vi "EDWARDS.vi"() -> ()   [LabVIEW 2022 SP3]
uses:
  Enum/Enum p4.ctl
  Variables globales/Variable glob generale.vi
  Variables globales/Variable glob Edwards.vi
  <vilib>/Instr/_visa.llb/VISA Configure Serial Port (Instr).vi
panel:
  out "Grappes TIC":cluster{"TIC":u8, "Voie":u8}[][](array[cluster])
  out "Sélection":bool[][](array[boolean])
  out "Port RS232 Edwards":refnum<visa-resource-name>[](array[refnum])
  out "Voies":i8[][](array[numeric]) min=1 max=6 step=1
  out "Données 1D":string[](array[string])
  out "Données Edwards":string[][](array[string])
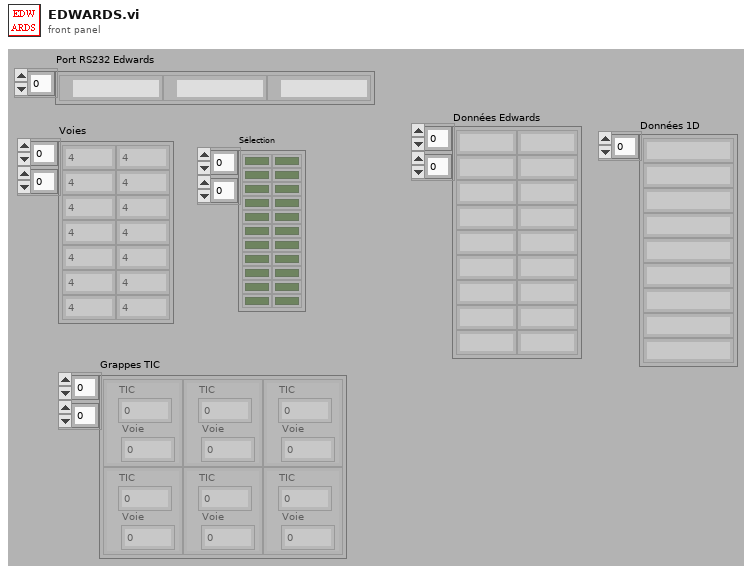
[diagram p1: front panel]
types:
  T1 = typedef "Enum p4.ctl" = enum16{"Init COM", "Lecture", "Grappes"}
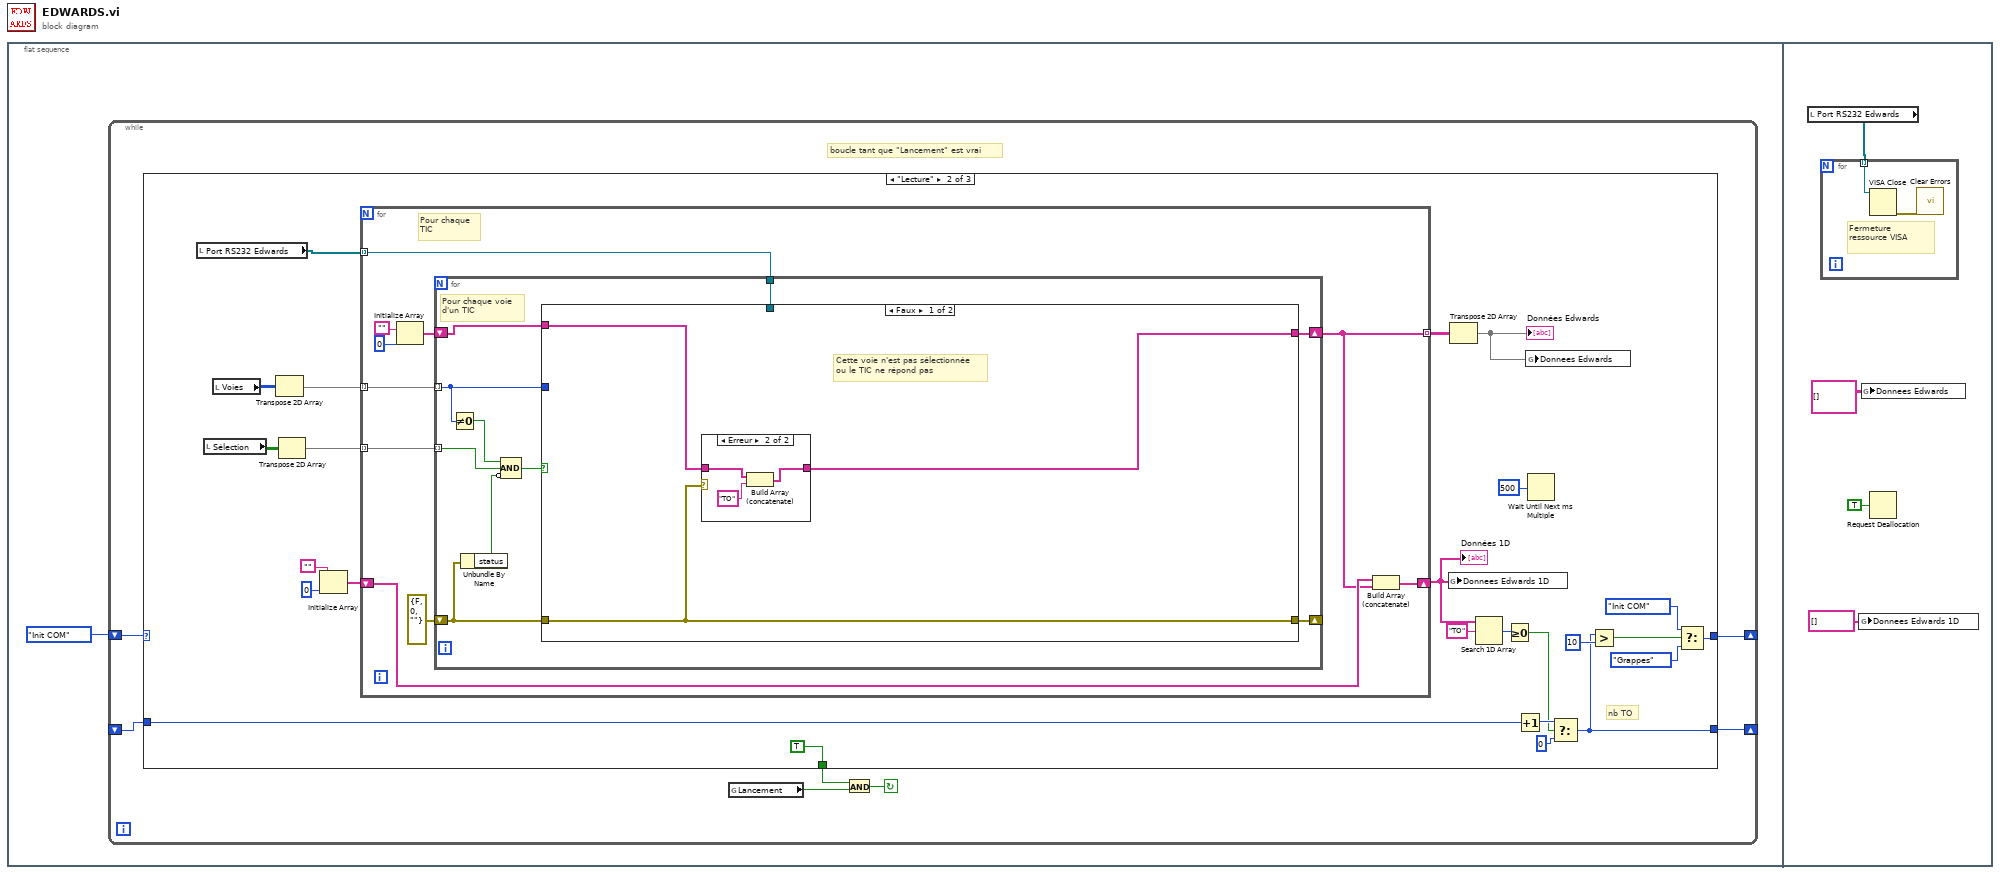
[diagram p0: block diagram]
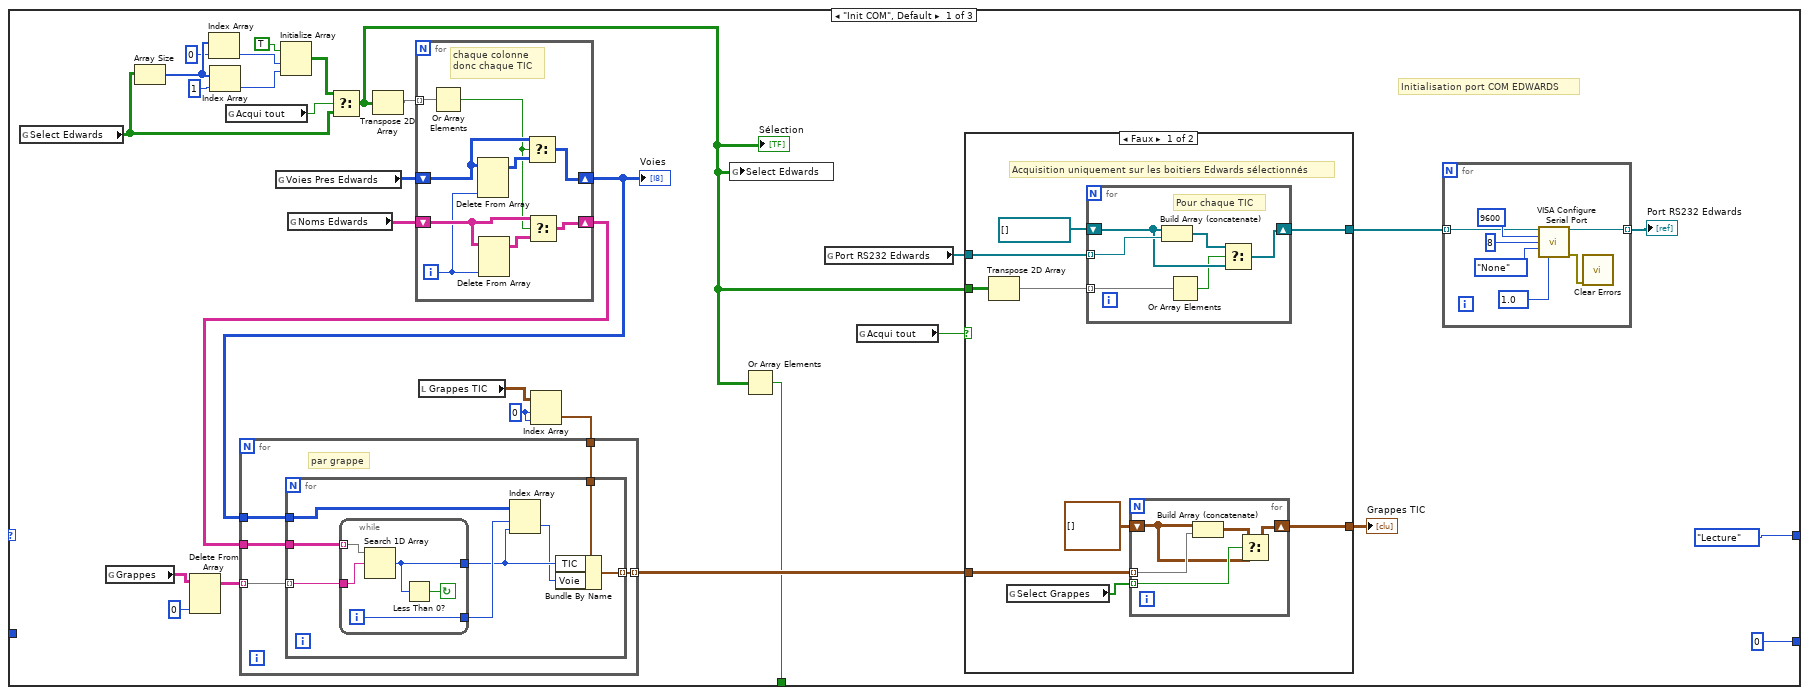
[diagram p2: hidden frame]
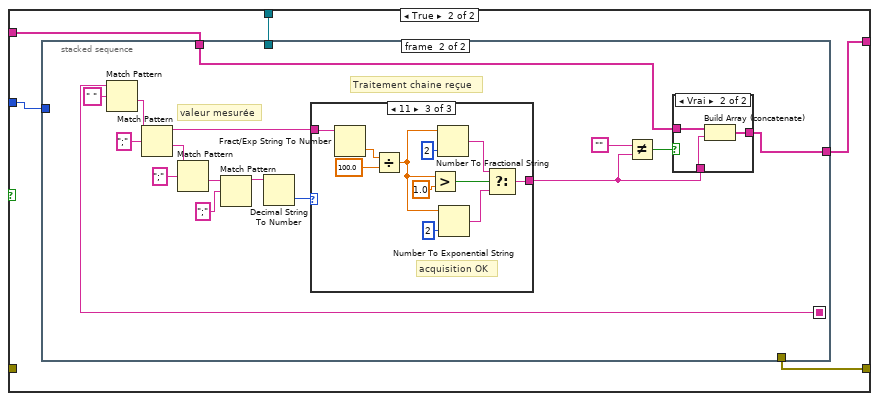
[diagram p5: hidden frame]
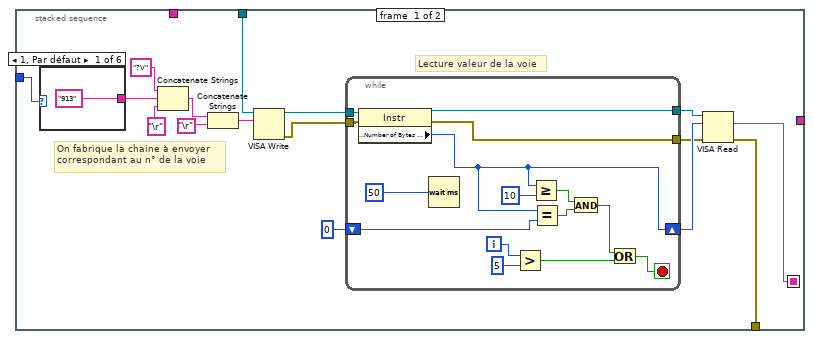
[diagram p6: hidden frame]
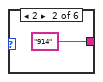
[diagram p7: hidden frame]
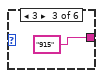
[diagram p8: hidden frame]
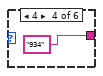
[diagram p9: hidden frame]
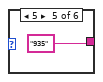
[diagram p10: hidden frame]
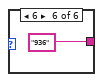
[diagram p11: hidden frame]
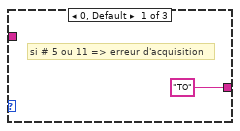
[diagram p13: hidden frame]
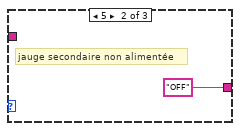
[diagram p14: hidden frame]
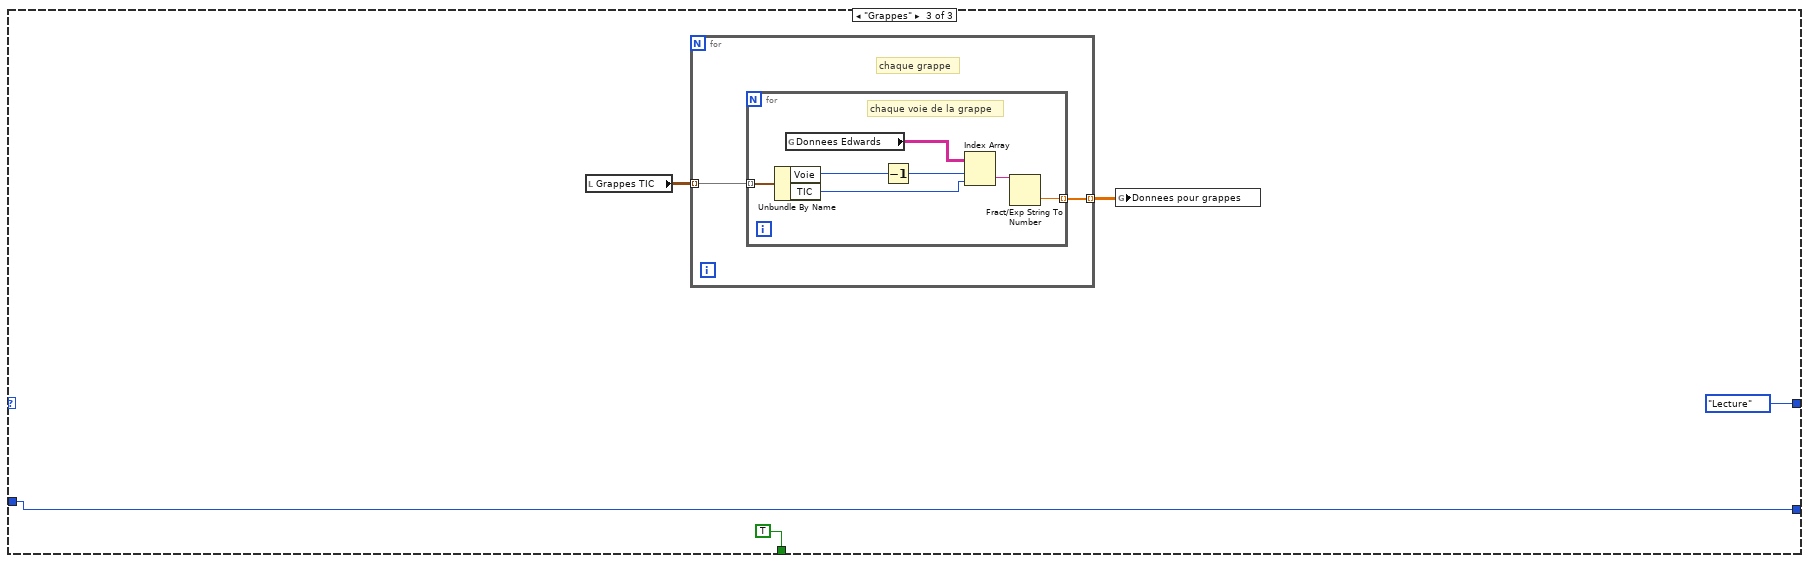
[diagram p15: hidden frame]
diagram:
  n1 = flat-sequence {
    frame #0 {
      n2 = while {
        shift-right: [w7] -> _
        shift-left: Enum_p4."Init COM" ("Énum") -> [w8]
        shift-right: [w6] -> _
        shift-left: _ -> [w5]
        stop <- w2 continue-if-true
        # "boucle tant que \"Lancement\" est vrai"
        n3 = case shown="\"Lecture\"" w8 {
          tunnel: [Enum_p4."Lecture" ("Énum") w104 Enum_p4."Lecture" ("Énum")] -> w7
          tunnel: [0 w100 w225] -> w6
          tunnel: w5 -> [_ w99 w225]
          tunnel: [w9 TRUE TRUE] -> w4
          frame "Init COM", Default {
            w24 = 0 ("indice (ligne)")
            # "Initialisation port COM EDWARDS"
            n4 = global read "Variable glob Edwards.vi" "Select Edwards"() -> (w19:bool[][])
            n5 = global read "Variable glob Edwards.vi" "Grappes"() -> (w25:string[][])
            n6 = Array Size(array=w19) -> (size(s)=w18:i32[])
            n7 = Delete From Array(array=w25, index (col)=0 ("indice désactivé (col)")) -> (array with subset deleted=w27:string[][])  [unwired: 2 in, 1 out]
            n8 = Index Array(array=w18, index=0 ("indice")) -> (element=w15:i32)
            n9 = Index Array(array=w18, index=1 ("indice")) -> (element=w14:i32)
            n10 = global read "Variable glob generale.vi" "Acqui tout"() -> (w20:bool)
            n11 = global read "Variable glob Edwards.vi" "Voies Pres Edwards"() -> (w30:i8[][])
            n12 = Initialize Array(TRUE, w15, w14) -> (w12:bool[][])
            n13 = global read "Variable glob Edwards.vi" "Noms Edwards"() -> (w31:string[][])
            n14 = Select(t=w12, s=w20, f=w19) -> (s? t:f=w10:bool[][])
            "Sélection" <- w10
            n15 = Transpose 2D Array(2D array=w10) -> (transposed array=w32:bool[][])
            n16 = for {
              tunnel: w32 -> [w65] mode=indexing
              shift-right: [w62] -> w23
              shift-left: w31 -> [w63]
              shift-right: [w57] -> w11
              shift-left: w30 -> [w60]
              i -> [w58]
              # "chaque colonne\ndonc chaque TIC"
              n17 = Or Array Elements(Boolean array=w65) -> (logical OR=w59:bool)
              n18 = Delete From Array(array=w60, index (col)=w58) -> (array with subset deleted=w61:i8[][])  [unwired: 2 in, 1 out]
              n19 = Delete From Array(array=w63, index (col)=w58) -> (array with subset deleted=w64:string[][])  [unwired: 2 in, 1 out]
              n20 = Select(t=w60, s=w59, f=w61) -> (s? t:f=w57:i8[][])
              n21 = Select(t=w63, s=w59, f=w64) -> (s? t:f=w62:string[][])
            }
            "Voies" <- w11
            n22 = local read "Grappes TIC"() -> (w29:cluster{"TIC":u8, "Voie":u8}[][])
            n23 = Index Array(array=w29, index (row)=w24, index (col)=w24) -> (element=w28:cluster{"TIC":u8, "Voie":u8})
            n24 = for {
              tunnel: w27 -> [w43] mode=indexing
              tunnel: w23 -> [w42]
              tunnel: w11 -> [w41]
              tunnel: [w40] -> w22 mode=indexing
              tunnel: w28 -> [w39]
              # "par grappe"
              n25 = for {
                tunnel: w43 -> [w48] mode=indexing
                tunnel: w42 -> [w49]
                tunnel: w41 -> [w47]
                tunnel: [w51] -> w40 mode=indexing
                tunnel: w39 -> [w50]
                n26 = while {
                  tunnel: w49 -> [w55] mode=indexing
                  tunnel: w48 -> [w56]
                  tunnel: [w54] -> w45
                  tunnel: [w52] -> w46
                  i -> [w52]
                  stop <- w53 continue-if-true
                  n27 = Search 1D Array(1D array=w55, element=w56) -> (index of element=w54:i32)  [unwired: 1 in]
                  n28 = Less Than 0?(x=w54) -> (x < 0?=w53:bool)
                }
                n29 = Index Array(array=w47, index (row)=w46, index (col)=w45) -> (element=w44:i8)
                n30 = Bundle By Name(cluster=w50, "TIC"=w45, "Voie"=w44) -> (w51:cluster{"TIC":u8, "Voie":u8})
              }
            }
            n31 = global write "Variable glob Edwards.vi" "Select Edwards"(w10) -> ()
            n32 = Or Array Elements(Boolean array=w10) -> (logical OR=w9:bool)
            n33 = global read "Variable glob Edwards.vi" "Port RS232 Edwards"() -> (w36:refnum<visa-resource-name>[])
            n34 = global read "Variable glob generale.vi" "Acqui tout"() -> (w37:bool)
            n35 = case shown="Faux" w37 {
              tunnel: [w73 w87] -> w35
              tunnel: w36 -> [w74 w87]
              tunnel: w10 -> [w71 _]
              tunnel: w22 -> [w67 w86]
              tunnel: [w66 w86] -> w21
              frame False {
                # "Acquisition uniquement sur les boitiers Edwards sélectionnés"
                n36 = Transpose 2D Array(2D array=w71) -> (transposed array=w70:bool[][])
                n37 = global read "Variable glob Edwards.vi" "Select Grappes"() -> (w69:bool[])
                n38 = for {
                  tunnel: w74 -> [w85] mode=indexing
                  tunnel: w70 -> [w80] mode=indexing
                  shift-right: [w83] -> w73
                  shift-left: refnum<visa-resource-name>[] [] -> [w82]
                  # "Pour chaque TIC"
                  n39 = Build Array (concatenate)(w82, w85) -> (w84:refnum<visa-resource-name>[])
                  n40 = Or Array Elements(Boolean array=w80) -> (logical OR=w81:bool)
                  n41 = Select(t=w84, s=w81, f=w82) -> (s? t:f=w83:refnum<visa-resource-name>[])
                }
                n42 = for {
                  tunnel: w69 -> [w79] mode=indexing
                  shift-right: [w75] -> w66
                  shift-left: cluster{"TIC":u8, "Voie":u8}[][] [] -> [w76]
                  tunnel: w67 -> [w78] mode=indexing
                  n43 = Build Array (concatenate)(w76, w78) -> (w77:cluster{"TIC":u8, "Voie":u8}[][])
                  n44 = Select(t=w77, s=w79, f=w76) -> (s? t:f=w75:cluster{"TIC":u8, "Voie":u8}[][])
                }
              }
              frame True {
                # "Acquisition sur l'ensemble des boitiers Edwards configurés"
              }
            }
            "Grappes TIC" <- w21
            n45 = for {
              tunnel: w35 -> [w90] mode=indexing
              tunnel: [w89] -> w38 mode=indexing
              w94 = u16 10 items=["1.0"=10, "1.5"=15, "2.0"=20] ("stop bits (10: 1 bit)")
              n46 = call-poly "VISA Configure Serial Port"("VISA resource name"=w90, "baud rate (9600)"=u32 9600, "data bits (8)"=u16 8, "parity (0:none)"=enum16{"None", "Odd", "Even", "Mark", "Space"}."None", "stop bits (10: 1 bit)"=w94) -> ("VISA resource name out"=w89:refnum<visa-resource-name>, "error out"=w88:errorcluster)  [unwired: 9 in]
              n47 = call <vilib>:"Clear Errors.vi"("error in (no error)"=w88) -> ()  [unwired: 5 in, 2 out]
            }
            "Port RS232 Edwards" <- w38
          }
          frame "Lecture" {
            # "nb TO"
            n48 = local read "Port RS232 Edwards"() -> (w113:refnum<visa-resource-name>[])
            n49 = local read "Sélection"() -> (w96:bool[][])
            n50 = local read "Voies"() -> (w112:i8[][])
            n51 = Transpose 2D Array(2D array=w112) -> (transposed array=w111:i8[][])
            n52 = Transpose 2D Array(2D array=w96) -> (transposed array=w110:bool[][])
            n53 = Initialize Array("", 0 ("taille de la dimension")) -> (w116:string[])
            n54 = for {
              tunnel: w111 -> [w129] mode=indexing
              tunnel: [w122] -> w119 mode=indexing
              tunnel: w110 -> [w125] mode=indexing
              tunnel: w113 -> [w121] mode=indexing
              shift-right: [w123] -> w109
              shift-left: w116 -> [w124]
              # "Pour chaque\nTIC"
              n55 = Initialize Array("", 0 ("taille de la dimension")) -> (w126:string[])
              n56 = for {
                tunnel: w129 -> [w136] mode=indexing
                tunnel: w121 -> [w139]
                shift-right: [w138] -> w122
                shift-left: w126 -> [w137]
                tunnel: w125 -> [w133] mode=indexing
                shift-right: [w135] -> _
                shift-left: errorcluster {"status"=FALSE, "code"=0, "source"=""} ("error out") -> [w131]
                # "Pour chaque voie\nd'un TIC"
                n57 = Not Equal To 0?(x=w136) -> (x != 0?=w134:bool)
                n58 = Unbundle By Name(w131) -> ("status"=w130:bool)
                n59 = Compound Arithmetic op=AND ("Opérateur arithmétique")(w134, w133, invert w130) -> (w132:bool)
                n60 = case shown="Faux" w132 {
                  tunnel: w136 -> [_ w150]
                  tunnel: w139 -> [_ w151]
                  tunnel: [w140 w148] -> w138
                  tunnel: w137 -> [w141 w149]
                  tunnel: [w142 w147] -> w135
                  tunnel: w131 -> [w142 _]
                  frame False {
                    # "Cette voie n'est pas sélectionnée\nou le TIC ne répond pas"
                    n61 = case shown="Erreur" w142 {
                      tunnel: w141 -> [w143 w146]
                      tunnel: [w143 w145] -> w140
                      frame No Error {
                      }
                      frame Error {
                        n62 = Build Array (concatenate)(w146, "TO") -> (w145:string[])
                      }
                    }
                  }
                  frame True {
                    n63 = stacked-sequence {
                      seq-local: [w154 _] -> [_ w194]
                      tunnel: w151 -> [w158 _]
                      tunnel: w150 -> [w155 _]
                      tunnel: w149 -> [_ w191]
                      tunnel: [_ w189] -> w148
                      tunnel: [w152 _] -> w147
                      frame #0 {
                        # "Lecture valeur de la voie"
                        # "On fabrique la chaine à envoyer\ncorrespondant au n° de la voie"
                        n64 = case shown="1, Par défaut" w155 {
                          tunnel: ["913" "914" "915" "934" "935" "936"] -> w156
                          frame 1, Default {
                          }
                          frame 2 {
                          }
                          frame 3 {
                          }
                          frame 4 {
                          }
                          frame 5 {
                          }
                          frame 6 {
                          }
                        }
                        n65 = Concatenate Strings("?V", w156, "\r") -> (w160:string)
                        n66 = Concatenate Strings(w160, "\r") -> (w157:string)
                        n67 = VISA Write(VISA resource name=w158, write buffer=w157) -> (VISA resource name out=w163:refnum<visa-resource-name>, error out=w153:errorcluster)  [unwired: 1 in, 1 out]
                        n68 = while {
                          tunnel: w163 -> [w188]
                          tunnel: [w181] -> w167
                          shift-right: [w180] -> w166
                          shift-left: 0 -> [w179]
                          tunnel: w153 -> [w175]
                          tunnel: [w174] -> w159
                          i -> [w186]
                          stop <- w187 stop-if-true
                          n69 = property class="Instr"(reference=w188, error in=w175) -> (reference out=w181:refnum<visa-resource-name>, error out=w174:errorcluster, "Serial Settings:Number of Bytes at Serial Port"=w180:u32)
                          n70 = Wait (ms)(milliseconds to wait=u32 50 ("attente (ms)")) -> ()  [unwired: 1 out]
                          n71 = Greater?(x=w186, y=5) -> (0:w184:bool)
                          n72 = Greater Or Equal?(x=w180, y=u32 10) -> (x >= y?=w177:bool)
                          n73 = Equal?(x=w180, y=w179) -> (x = y?=w178:bool)
                          n74 = And(x=w177, y=w178) -> (x .and. y?=w176:bool)
                          n75 = Or(x=w176, y=w184) -> (x .or. y?=w187:bool)
                        }
                        n76 = VISA Read(VISA resource name=w167, byte count=w166, error in (no error)=w159) -> (read buffer=w154:string, error out=w152:errorcluster)  [unwired: 2 out]
                      }
                      frame #1 {
                        # "valeur mesurée"
                        # "Traitement chaine reçue"
                        n77 = Match Pattern(string=w194, regular expression=" " ("expression régulière")) -> (after substring=w196:string)  [unwired: 1 in, 3 out]
                        n78 = Match Pattern(string=w196, regular expression=";" ("expression régulière")) -> (before substring=w200:string, after substring=w199:string)  [unwired: 1 in, 2 out]
                        n79 = Match Pattern(string=w199, regular expression=";" ("expression régulière")) -> (after substring=w201:string)  [unwired: 1 in, 3 out]
                        n80 = Match Pattern(string=w201, regular expression=";" ("expression régulière")) -> (before substring=w203:string)  [unwired: 1 in, 3 out]
                        n81 = Decimal String To Number(string=w203) -> (number=w204:i32)  [unwired: 2 in, 1 out]
                        n82 = case shown="11" w204 {
                          tunnel: w200 -> [_ _ w221]
                          tunnel: ["TO" "OFF" w215] -> w190
                          frame 0, Default {
                            # "si # 5 ou 11 => erreur d'acquisition"
                          }
                          frame 5 {
                            # "jauge secondaire non alimentée"
                          }
                          frame 11 {
                            # "acquisition OK"
                            n83 = Fract/Exp String To Number(string=w221) -> (number=w220:dbl)  [unwired: 3 in, 1 out]
                            n84 = Divide(x=w220, y=100.0) -> (x/y=w212:dbl)
                            n85 = Greater?(x=w212, y=1.0) -> (0:w213:bool)
                            n86 = Number To Fractional String(number=w212, precision (6)=i16 2 ("précision (6)")) -> (F-format string=w216:string)  [unwired: 2 in]
                            n87 = Number To Exponential String(number=w212, precision (6)=i16 2 ("précision (6)")) -> (E-format string=w211:string)  [unwired: 2 in]
                            n88 = Select(t=w216, s=w213, f=w211) -> (s? t:f=w215:string)
                          }
                        }
                        n89 = Not Equal?(x="", y=w190) -> (x != y?=w193:bool)
                        n90 = case shown="Vrai" w193 {
                          tunnel: w191 -> [w205 w208]
                          tunnel: w190 -> [_ w207]
                          tunnel: [w205 w206] -> w189
                          frame False {
                          }
                          frame True {
                            n91 = Build Array (concatenate)(w208, w207) -> (w206:string[])
                          }
                        }
                      }
                    }
                  }
                }
              }
              n92 = Build Array (concatenate)(w124, w122) -> (w123:string[])
            }
            "Données 1D" <- w109
            n93 = global write "Variable glob Edwards.vi" "Donnees Edwards 1D"(w109) -> ()
            n94 = Transpose 2D Array(2D array=w119) -> (transposed array=w114:string[][])
            "Données Edwards" <- w114
            n95 = Search 1D Array(1D array=w109, element="TO" ("élément")) -> (index of element=w107:i32)  [unwired: 1 in]
            n96 = Greater Or Equal To 0?(x=w107) -> (x >= 0?=w97:bool)
            n97 = Increment(x=w99) -> (x+1=w101:i32)
            n98 = global write "Variable glob Edwards.vi" "Donnees Edwards"(w114) -> ()
            n99 = Wait Until Next ms Multiple(millisecond multiple=u32 500 ("n millisecondes")) -> ()  [unwired: 1 out]
            n100 = Select(t=w101, s=w97, f=0 ("cas faux")) -> (s? t:f=w100:i32)
            n101 = Greater?(x=w100, y=10) -> (0:w98:bool)
            n102 = Select(t=Enum_p4."Init COM" ("Énum"), s=w98, f=Enum_p4."Grappes" ("Énum")) -> (s? t:f=w104:T1)
          }
          frame "Grappes" {
            n103 = local read "Grappes TIC"() -> (w224:cluster{"TIC":u8, "Voie":u8}[][])
            n104 = for {
              tunnel: w224 -> [w228] mode=indexing
              tunnel: [w227] -> w223 mode=indexing
              # "chaque grappe"
              n105 = for {
                tunnel: w228 -> [w235] mode=indexing
                tunnel: [w230] -> w227 mode=indexing
                # "chaque voie de la grappe"
                n106 = Unbundle By Name(w235) -> ("Voie"=w233:u8, "TIC"=w232:u8)
                n107 = global read "Variable glob Edwards.vi" "Donnees Edwards"() -> (w234:string[][])
                n108 = Decrement(x=w233) -> (x-1=w229:u8)
                n109 = Index Array(array=w234, index (row)=w229, index (col)=w232) -> (element=w231:string)
                n110 = Fract/Exp String To Number(string=w231) -> (number=w230:dbl)  [unwired: 3 in, 1 out]
              }
            }
            n111 = global write "Variable glob Edwards.vi" "Donnees pour grappes"(w223) -> ()
          }
        }
        n112 = global read "Variable glob generale.vi" "Lancement"() -> (w3:bool)
        n113 = And(x=w4, y=w3) -> (x .and. y?=w2:bool)
      }
    }
    frame #1 {
      n114 = local read "Port RS232 Edwards"() -> (w236:refnum<visa-resource-name>[])
      n115 = for {
        tunnel: w236 -> [w240] mode=indexing
        # "Fermeture\nressource VISA"
        n116 = VISA Close(VISA resource name=w240) -> (error out=w241:errorcluster)  [unwired: 1 in]
        n117 = call <vilib>:"Clear Errors.vi"("error in (no error)"=w241) -> ()  [unwired: 5 in, 2 out]
      }
      n118 = global write "Variable glob Edwards.vi" "Donnees Edwards 1D"(string[] [] ("Données Edwards 1D")) -> ()
      n119 = global write "Variable glob Edwards.vi" "Donnees Edwards"(string[][] [] ("Données Edwards")) -> ()
      n120 = Request Deallocation(TRUE ("flag")) -> ()
    }
  }
